vi "Declare OpModes.vi"() -> (3 "OpModes":T1)   [LabVIEW 2023]
doc: "Template code for declaring the Autonomous OpModes, TeleOperated OpModes, and Utility/Test OpModes that will be displayed in the Driver Station.\nGrow the array node to add as many as are needed."
uses:
  <vilib>/MRC/MrcLib/VIs/Robot Framework/DS OpModes.ctl
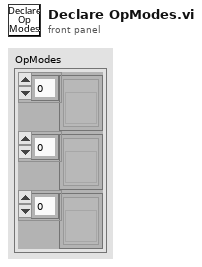
[diagram p1: front panel]
types:
  T1 = typedef "DS OpModes.ctl" = cluster{"Autos":refnum<vi>[], "Teles":refnum<vi>[], "Utilities":refnum<vi>[]}
  T2 = cluster{refnum<vi>[], refnum<vi>[], refnum<vi>[]}
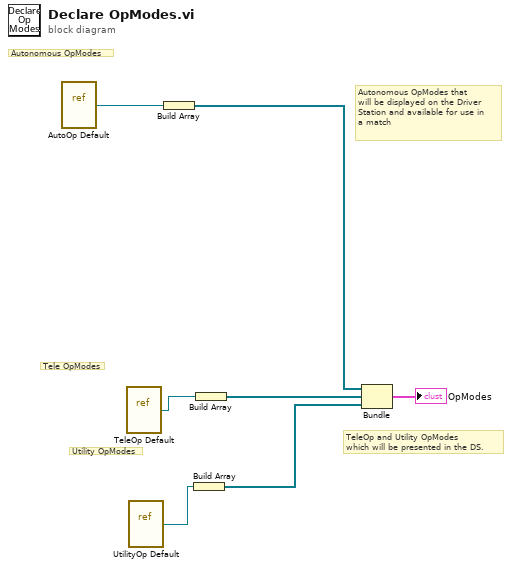
[diagram p0: block diagram]
diagram:
  # "TeleOp and Utility OpModes\nwhich will be presented in the DS."
  # "Autonomous OpModes that\nwill be displayed on the Driver\nStation and available for use in\na match"
  # "Utility OpModes"
  # "Tele OpModes"
  # "Autonomous OpModes"
  n1 = vi-ref "AutoOp Default.vi"() -> (w4:refnum<vi>)
  n2 = vi-ref "TeleOp Default.vi"() -> (w3:refnum<vi>)
  n3 = vi-ref "UtilityOp Default.vi"() -> (w2:refnum<vi>)
  n4 = Build Array(w4) -> (w5:refnum<vi>[])
  n5 = Build Array(w2) -> (w6:refnum<vi>[])
  n6 = Build Array(w3) -> (w7:refnum<vi>[])
  n7 = Bundle(w5, w7, w6) -> (→"OpModes":T2)  [unwired: 1 in]
